vi "Simulation.vi"() -> (3 "Measurement_Data out":T1)   [LabVIEW 2026]
uses:
  Measurement_Data.ctl
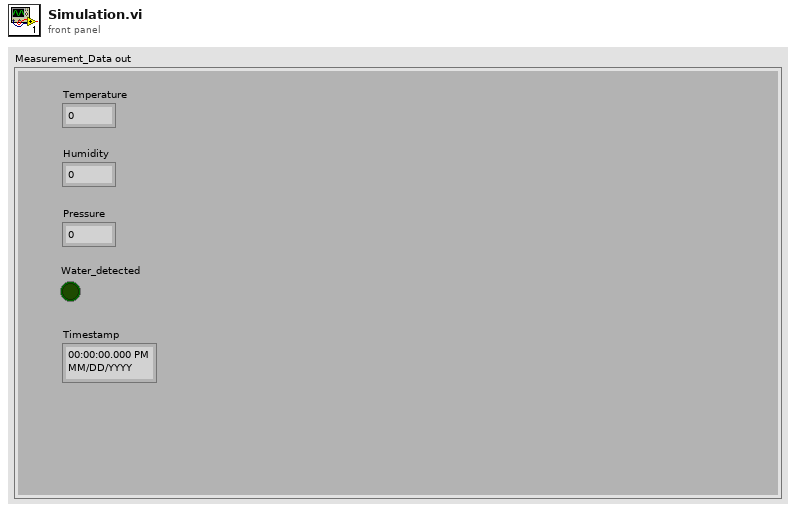
[diagram p1: front panel]
types:
  T1 = typedef "Measurement_Data.ctl" = cluster{"Temperature":dbl, "Humidity":dbl, "Pressure":dbl, "Water_detected":bool, "Timestamp":timestamp}
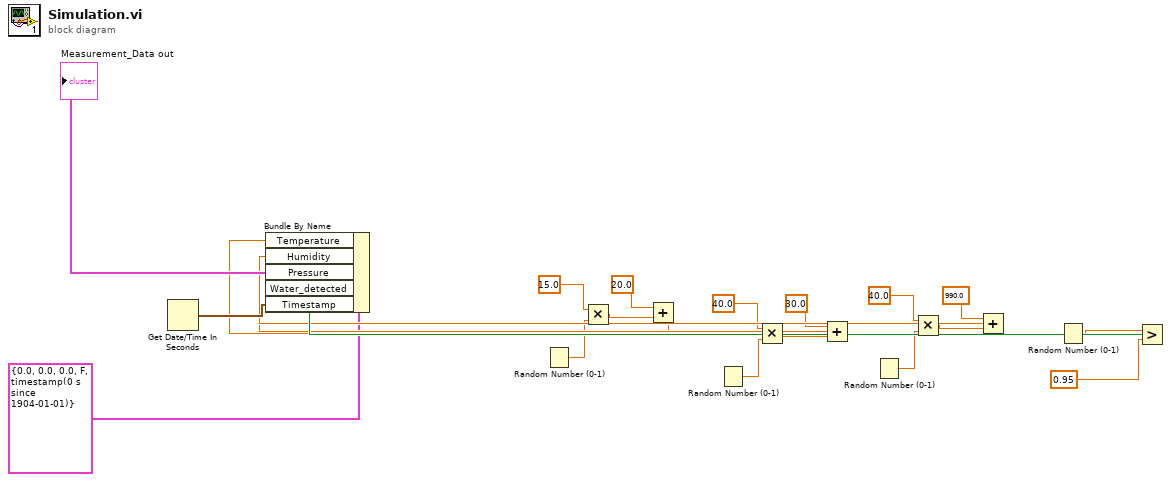
[diagram p0: block diagram]
diagram:
  n1 = Get Date/Time In Seconds() -> (seconds since 1Jan1904=w21:timestamp)
  n2 = Random Number (0-1)() -> (number: 0 to 1=w2:dbl)
  n3 = Multiply(x=15.0, y=w2) -> (x*y=w4:dbl)
  n4 = Add(x=20.0, y=w4) -> (x+y=w6:dbl)
  n5 = Random Number (0-1)() -> (number: 0 to 1=w7:dbl)
  n6 = Multiply(x=40.0, y=w7) -> (x*y=w9:dbl)
  n7 = Add(x=30.0, y=w9) -> (x+y=w11:dbl)
  n8 = Random Number (0-1)() -> (number: 0 to 1=w12:dbl)
  n9 = Multiply(x=40.0, y=w12) -> (x*y=w14:dbl)
  n10 = Add(x=990.0, y=w14) -> (x+y=w16:dbl)
  n11 = Random Number (0-1)() -> (number: 0 to 1=w17:dbl)
  n12 = Greater?(x=w17, y=0.95) -> (0:w19:bool)
  n13 = Bundle By Name(cluster=T1 {"Temperature"=0.0, "Humidity"=0.0, "Pressure"=0.0, "Water_detected"=FALSE, "Timestamp"=timestamp(0 s since 1904-01-01)} ("Measurement_Data"), "Temperature"=w6, "Humidity"=w11, "Pressure"=w16, "Water_detected"=w19, "Timestamp"=w21) -> (→"Measurement_Data out":T1)
